vi "CreateClass.vi"(0 "ClassWriterGOOP300.lvclass":refnum<class "ClassWriterGOOP300.lvclass">, 1 "ProjectTreePosition(String or Project Item Ref)":variant, 2 "CreateClassData":T1, 5 "error in (no error)":errorcluster, 6 "KeepLvClassRefOpen(False)":bool, 7 "HeaderToApply (take from VIRef or /use 2D-8bit header, Ignored if not wired)":variant) -> (14 "ClassWriterGOOP300.lvclass":refnum<class "ClassWriterGOOP300.lvclass">, 15 "LVClassLibraryRefnum":refnum<vi>, 16 "TemplateVersionUsed":string, 19 "error out":errorcluster)   [LabVIEW 2020, in "ClassWriterGOOP300.lvclass"]
uses:
  ClassWriterGOOP300.lvclass
  Provider_BaseClassInterface/CreateClassData.ctl
  Common/LvClass_class/GDSLvCLass_ClassSettingsType.ctl
  Common/LvClass_class/GDSLvClass_PlugIn.ctl
  Common/LvClass_class/GDSLvClass_PlugInTypes.ctl
  Provider_EndevoGOOP400/EndevoG4ProviderName.ctl
  EndevoProviderName.ctl
  Provider_BaseClassInterface/ClassWriter_class/ClassWriter.lvclass
  Provider_LvNativeClass/ClassWriterNative_class/ClassWriterNative.lvclass
  Provider_EndevoGOOP400/ClassWriterGOOP400_class/ClassWriterGOOP400.lvclass
  Common/InterfaceLibrary/InterfaceLibrary.lvlib
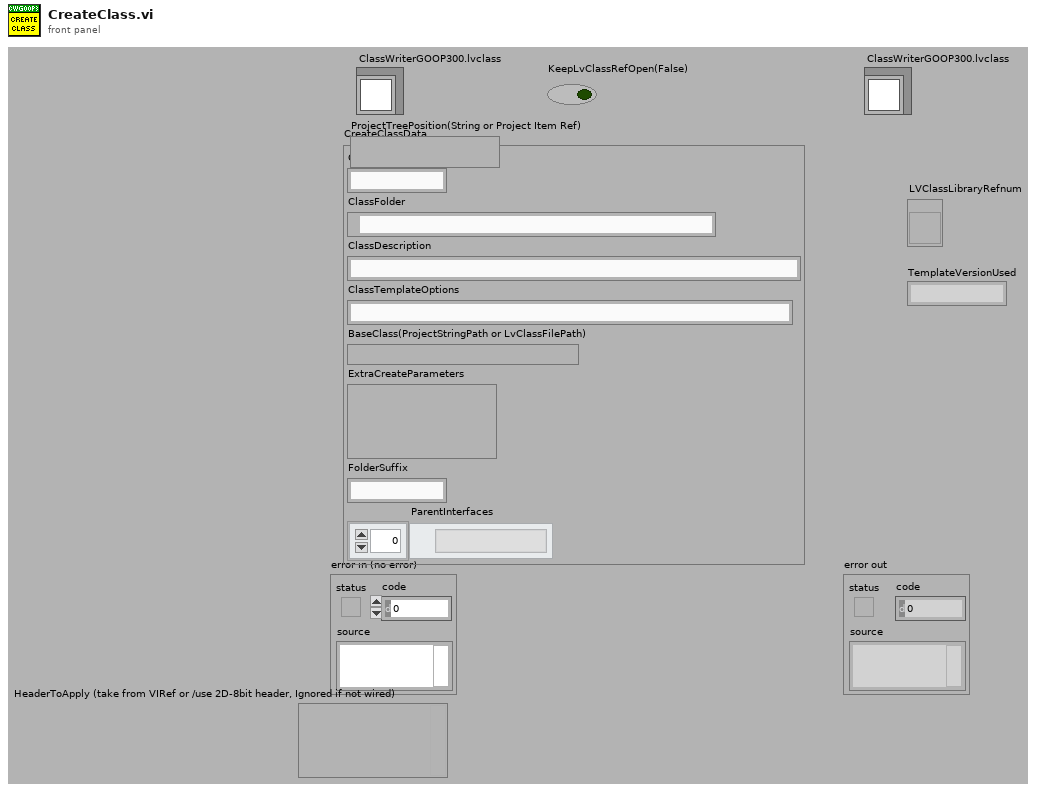
[diagram p1: front panel]
types:
  T1 = typedef "ClassWriter.lvclass/CreateClassData.ctl" = cluster{"ClassName":string, "ClassFolder":path, "ClassDescription":string, "ClassTemplateOptions":string, "BaseClass(ProjectStringPath or LvClassFilePath)":variant, "ExtraCreateParameters":variant, "FolderSuffix":string, "ParentInterfaces":path[]}
  T2 = typedef "GDSLvCLass_ClassSettingsType.ctl" = cluster{"ClassProviderName":string, "ClassTemplateUsed":string, "ClassTemplateVersion":string, "ClassDescription":string, "PlugIns":T3[], "ConnectorPanePattern":string}
  T3 = typedef "GDSLvClass_PlugIn.ctl" = cluster{"Type":T4, "ID":string, "Version":string, "Path":path, "Name":string, "Data":variant}
  T4 = typedef "GDSLvClass_PlugInTypes.ctl" = enum16{"DesignPattern", "MethodTypes"}
  T5 = cluster{"SubClass":bool, "ClassTemplateFiles":path[], "ClassName":string, "ClassFolder":path, "VIs":refnum<vi>[], "TemplateFolder":path, "ViSubDirs":string[], "TemplateName":string, "BaseClassFolder":path, "RootBaseClassFolder":path, "LvClassPath":path, "ClassRefnum":refnum<vi>, "ProjectRefnum":refnum<vi>, "LvClassFolderPath":path, "BaseClassName":string, "ClassItems":refnum<vi>[], "ViLocked":bool[], "ProjectItemOwner":refnum<vi>, "DeleteFiles":path[], "VIsBefore":refnum<vi>[], "BaseClassPath":path, "BaseConstructorBase":path, "TemplBaseConstructorBase":path, "TemplatePath":path, "TemplateVersion":string, "TemplateParentClass":refnum<vi>, "App":refnum<vi>, "Parent Class":refnum<vi>, "ParentVIs":refnum<vi>[], "TempClass":refnum<vi>, "TemplateParentName":string, "llb":bool, "ClassSettings":T2}
  T6 = typedef "EndevoG4ProviderName.ctl" = enum16{"EndevoGOOP400"}
  T7 = typedef "EndevoProviderName.ctl" = enum16{"EndevoGOOP300"}
  T8 = enum32{"invalid scope", "public", "private", "protected"}
  T9 = enum16{"Share clones between instances", "Preallocate clone for each instance"}
  T10 = enum32{"invalid lock state", "Not Locked", "Locked (No Password)", "Password-protected"}
  T11 = typedef "ClassWriter.lvclass/TemplateSettings.ctl" = cluster{"CommonClassTemplate":bool, "DynamicDispatch":enum8{"False", "True", "Mixed"}, "MustOverride":enum8{"False", "True", "Mixed"}, "MustCallParent":enum8{"False", "True", "Mixed"}, "OnlyNormalMethod":bool, "OnlyPublic":bool}
  T12 = typedef "Scripting_ConnectorPanePatternType.ctl" = u16
  T13 = typedef "GOOP400_Options.ctl" = cluster{"FlatFolderStructure":bool}
  T14 = typedef "imagedata.ctl" = cluster{"image type":i32, "image depth":i32, "image":u8[], "mask":u8[], "colors":u32[], "Rectangle":cluster{"left":i16, "top":i16, "right":i16, "bottom":i16}}
  T15 = typedef "Librarian File Info Out.ctl" = cluster{"creation date":u32, "last mod date":u32, "type":string, "creator":string, "LV version":i32, "size":i32, "top level":bool}
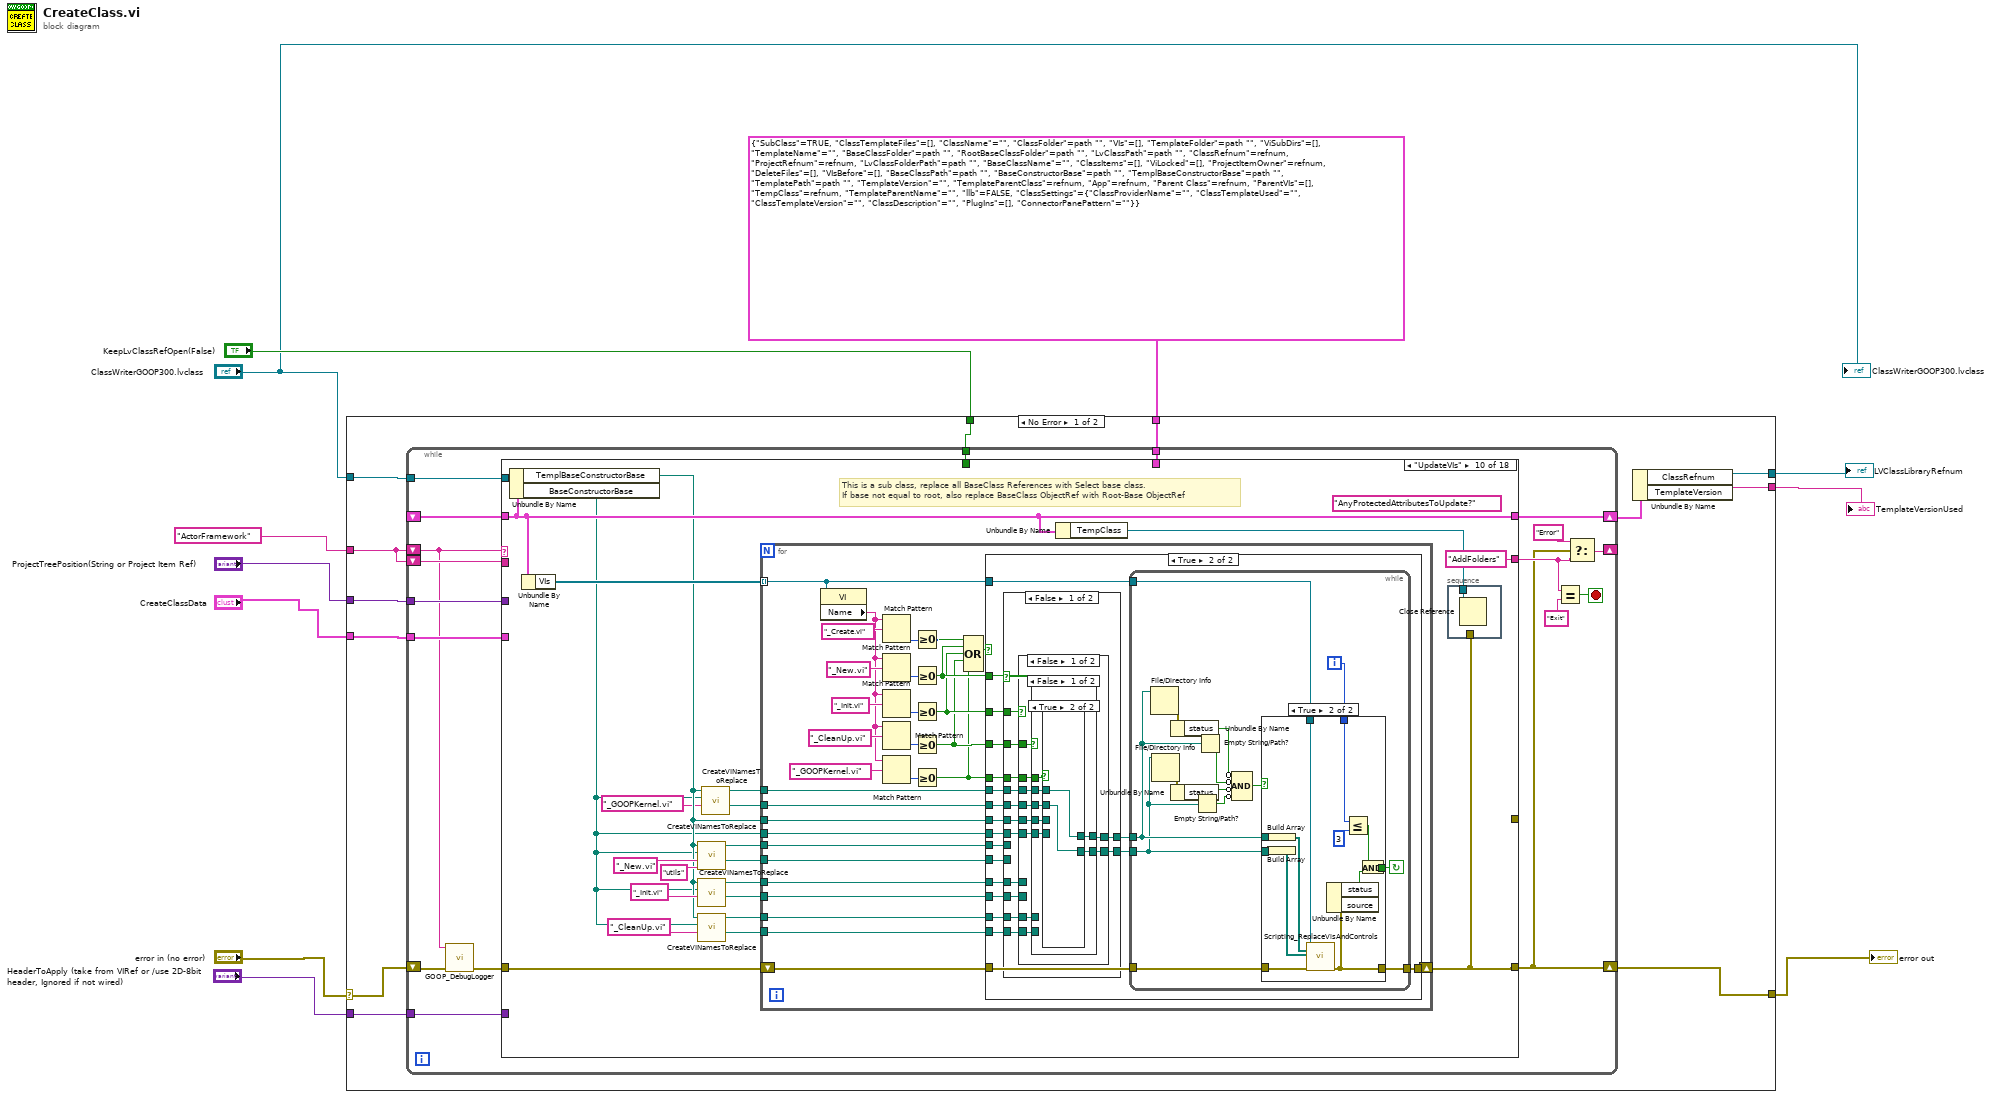
[diagram p0: block diagram]
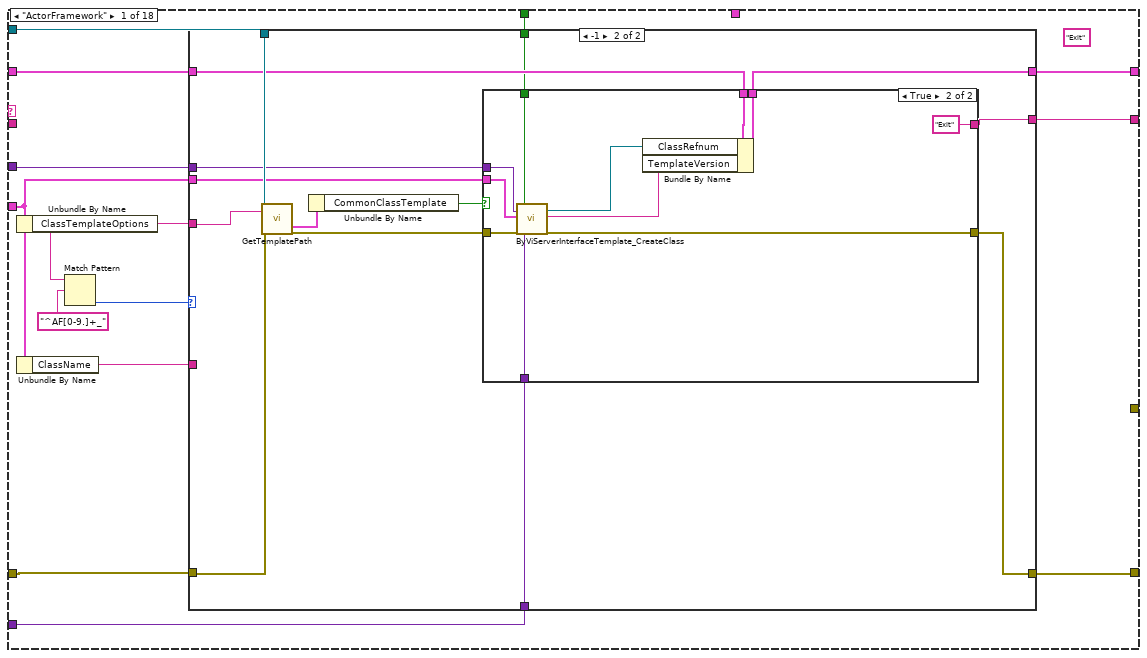
[diagram p2: hidden frame]
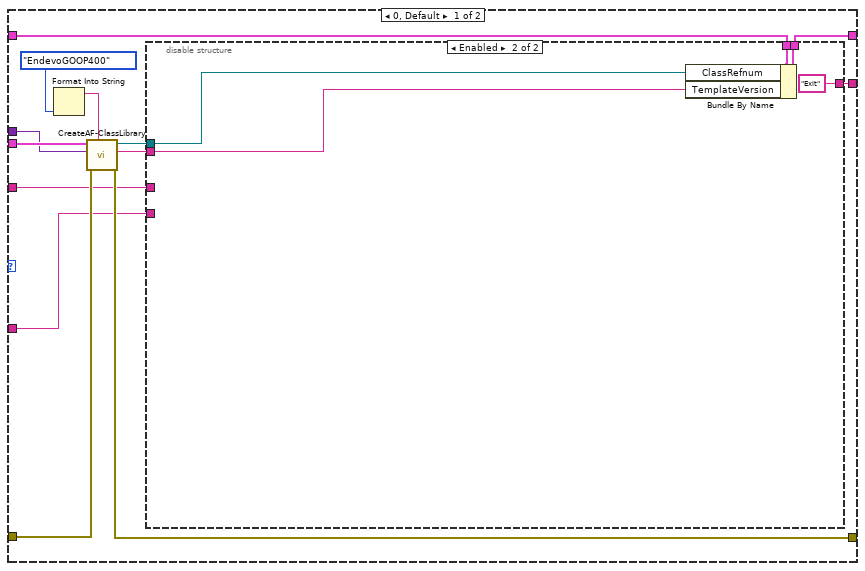
[diagram p3: hidden frame]
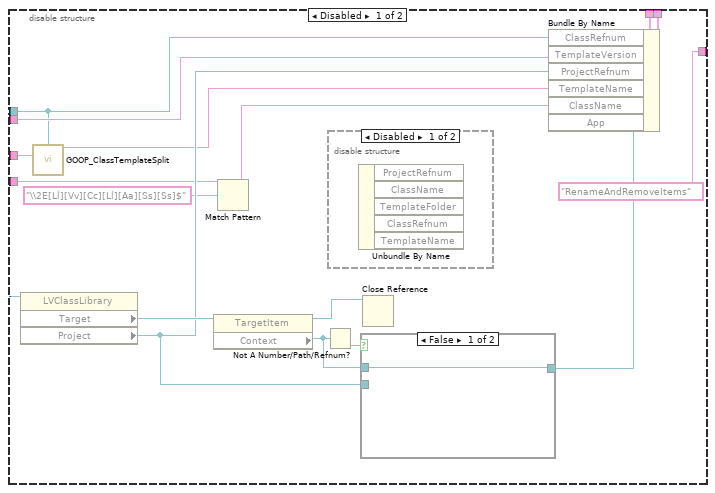
[diagram p4: hidden frame]
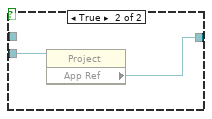
[diagram p6: hidden frame]
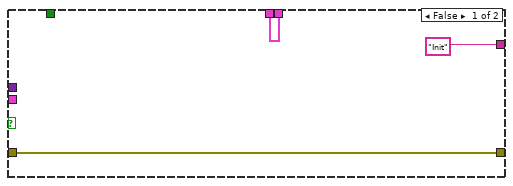
[diagram p7: hidden frame]
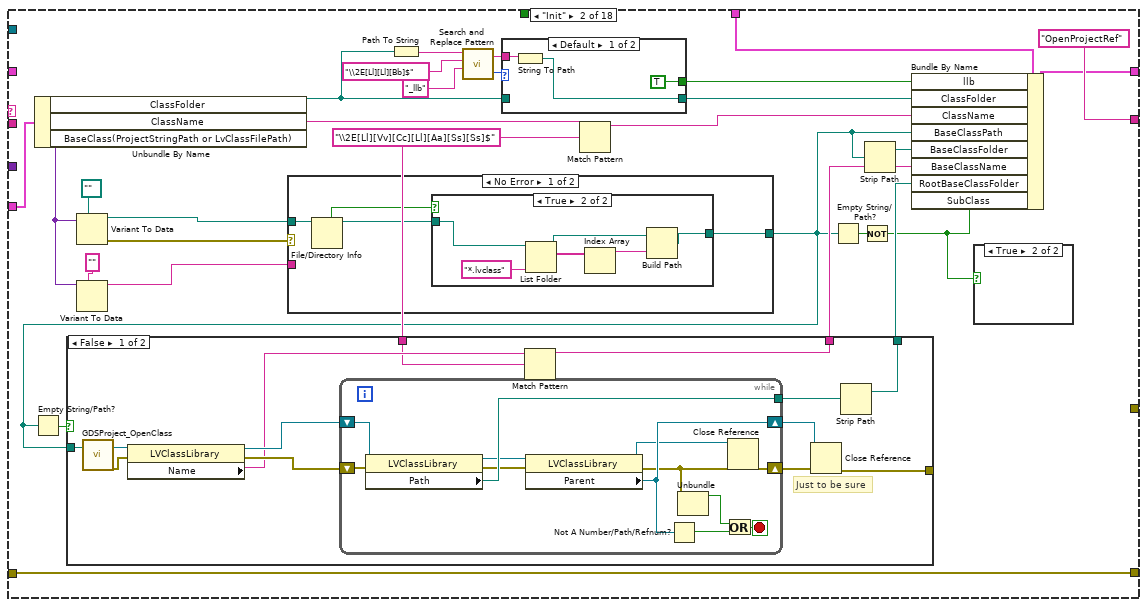
[diagram p8: hidden frame]
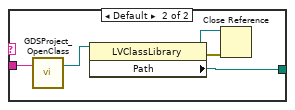
[diagram p14: hidden frame]
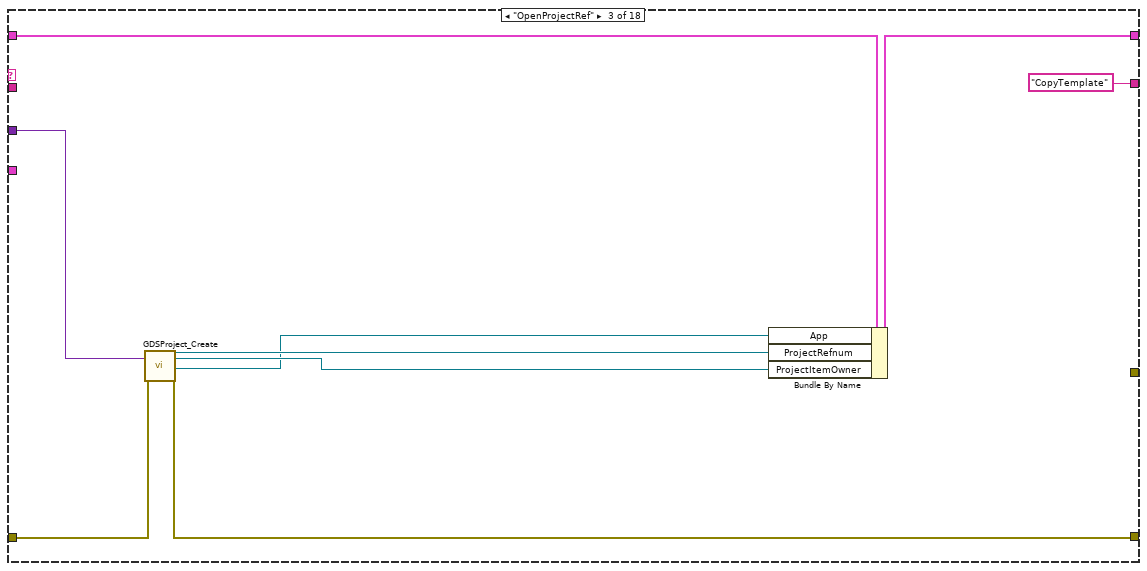
[diagram p15: hidden frame]
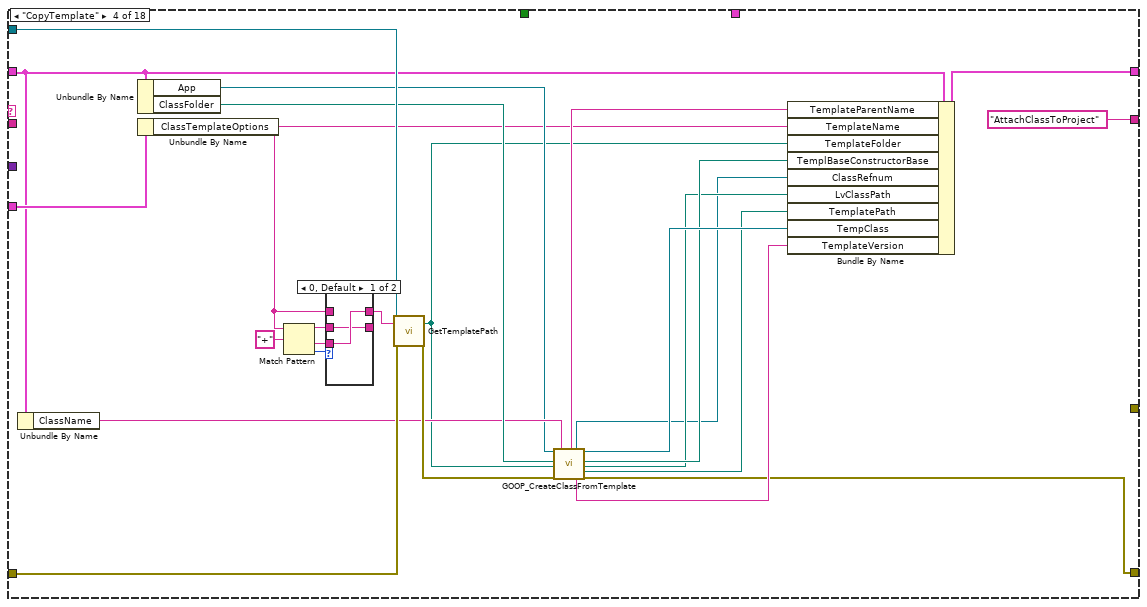
[diagram p16: hidden frame]
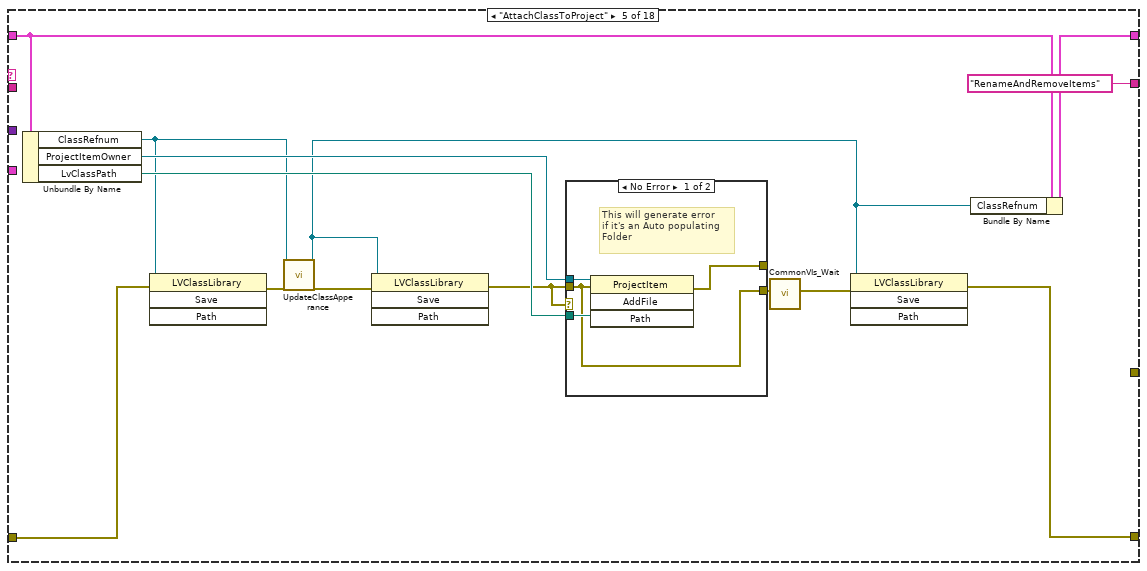
[diagram p18: hidden frame]
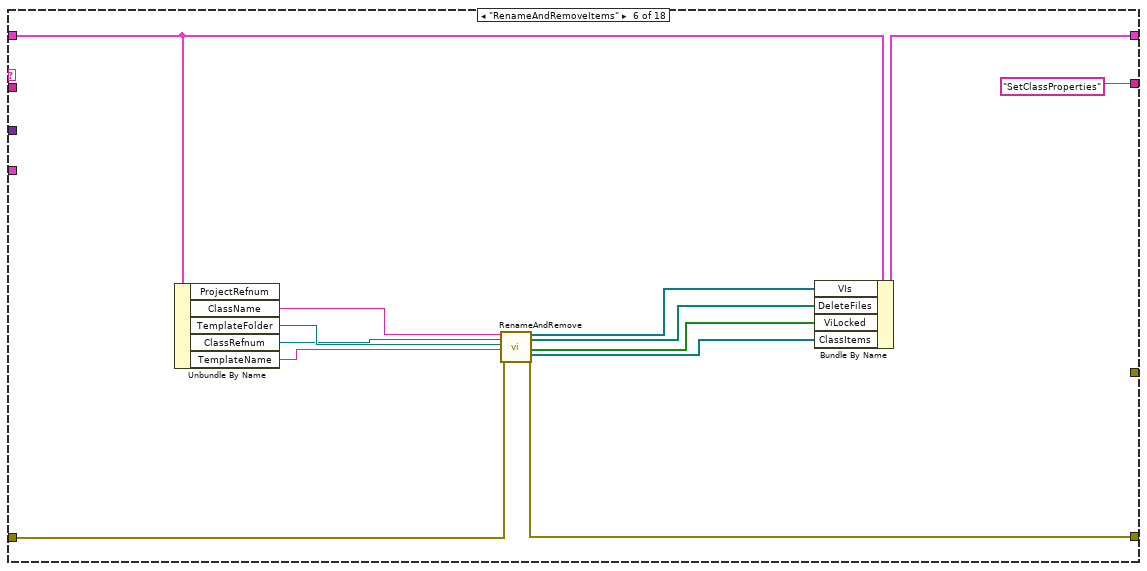
[diagram p20: hidden frame]
diagram:
  n1 = case shown="No Error" "error in (no error)" {
    selector: "error in (no error)" -> [w13 w824]
    tunnel: [w23 w824] -> w11
    tunnel: "ProjectTreePosition(String or Project Item Ref)" -> [w22 _]
    tunnel: "CreateClassData" -> [w21 _]
    tunnel: "ClassWriterGOOP300.lvclass" -> [w20 _]
    tunnel: "HeaderToApply (take from VIRef or /use 2D-8bit header, Ignored if not wired)" -> [w19 _]
    tunnel: "KeepLvClassRefOpen(False)" -> [w18 _]
    tunnel: [w17 _] -> w5
    tunnel: [w16 _] -> w4
    tunnel: T5 {"SubClass"=TRUE, "ClassTemplateFiles"=[], "ClassName"="", "ClassFolder"=path "", "VIs"=[], "TemplateFolder"=path "", "ViSubDirs"=[], "TemplateName"="", "BaseClassFolder"=path "", "RootBaseClassFolder"=path "", "LvClassPath"=path "", "ClassRefnum"=refnum, "ProjectRefnum"=refnum, "LvClassFolderPath"=path "", "BaseClassName"="", "ClassItems"=[], "ViLocked"=[], "ProjectItemOwner"=refnum, "DeleteFiles"=[], "VIsBefore"=[], "BaseClassPath"=path "", "BaseConstructorBase"=path "", "TemplBaseConstructorBase"=path "", "TemplatePath"=path "", "TemplateVersion"="", "TemplateParentClass"=refnum, "App"=refnum, "Parent Class"=refnum, "ParentVIs"=[], "TempClass"=refnum, "TemplateParentName"="", "llb"=FALSE, "ClassSettings"={"ClassProviderName"="", "ClassTemplateUsed"="", "ClassTemplateVersion"="", "ClassDescription"="", "PlugIns"=[], "ConnectorPanePattern"=""}} ("output cluster") -> [w15 _]
    tunnel: "ActorFramework" -> [w12 _]
    frame No Error {
      n2 = while {
        shift-right: [w33] -> w23
        shift-left: w13 -> [w26]
        shift-right: [w37] -> _
        shift-left: w12 -> [w24]
        shift-right: [w40] -> w14
        shift-left: _ -> [w41]
        tunnel: w15 -> [w35]
        tunnel: w22 -> [w32]
        tunnel: w21 -> [w31]
        tunnel: w20 -> [w30]
        shift-left: w12 -> [w29]
        tunnel: w19 -> [w28]
        tunnel: w18 -> [w27]
        stop <- w38 stop-if-true
        n3 = call "GOOP_DebugLogger.vi"("error in (no error)"=w26, "State"=w24) -> ("error out"=w25:errorcluster)  [unwired: 7 in, 2 out]
        n4 = case shown="\"UpdateVIs\"" w24 {
          selector: w24 -> [_ _ _ _ _ _ _ _ _ _ _ _ _ _ _ _ _ w775]
          tunnel: w41 -> [w55 _ w203 w214 w245 w260 w278 w328 w350 w364 w497 w554 w591 w643 w669 w680 w728 w759]
          tunnel: [w54 w146 w202 w213 w244 w262 w267 w328 w351 w364 w497 w554 w591 w643 w669 w680 w728 w759] -> w40
          tunnel: w25 -> [w50 w149 w201 w226 w239 w257 w279 w321 w347 w376 w518 w566 w592 w647 w668 w681 w731 w776]
          tunnel: [w49 w149 w199 w211 w235 w258 w270 w318 w333 w362 w498 w567 w593 w648 w667 w681 w714 w772] -> w33
          tunnel: [w53 "OpenProjectRef" "CopyTemplate" "AttachClassToProject" "RenameAndRemoveItems" "SetClassProperties" "UpdateIcons" w330 "UpdateVIs" ("t") "AddFolders" "AddFolders" w553 "PlaceRefInAttribute" "PlaceRefInAttribute" "ReentrantDestructor?" w685 "CloseRefs" "Exit"] -> w34
          tunnel: w35 -> [_ w142 _ _ _ _ _ _ _ _ _ _ _ _ _ _ _ _]
          tunnel: w32 -> [w48 _ w200 _ _ _ _ _ _ _ _ _ _ _ _ _ _ _]
          tunnel: w31 -> [w46 w141 _ w228 _ _ w285 _ _ _ _ w552 _ _ _ _ w733 _]
          tunnel: w30 -> [w44 _ _ w227 _ _ _ w315 _ _ _ _ _ w649 _ _ _ _]
          tunnel: w29 -> [_ _ _ _ _ _ _ _ _ _ _ _ _ _ _ _ _ w771]
          tunnel: w28 -> [w42 _ _ _ _ _ _ w326 _ _ _ _ _ _ _ _ _ _]
          tunnel: w27 -> [w43 _ _ _ _ _ _ _ _ _ _ _ _ _ _ _ _ w767]
          tunnel: [_ _ _ _ _ _ _ _ _ _ _ _ _ _ _ _ _ w765] -> _
          frame "ActorFramework" {
            (unwired) "Exit"
            n5 = Unbundle By Name(w46) -> ("ClassTemplateOptions"=w47:string)
            n6 = Unbundle By Name(w46) -> ("ClassName"=w45:string)
            n7 = Match Pattern(string=w47, regular expression="^AF[0-9.]+_") -> (offset past match=w51:i32)  [unwired: 1 in, 3 out]
            n8 = case shown="-1" w51 {
              tunnel: w55 -> [w68 w100]
              tunnel: [w67 w99] -> w54
              tunnel: [w59 w106] -> w53
              tunnel: w46 -> [w65 w96]
              tunnel: w50 -> [w64 w104]
              tunnel: [w63 w101] -> w49
              tunnel: w48 -> [w60 w97]
              tunnel: w47 -> [w57 w103]
              tunnel: w45 -> [w56 _]
              tunnel: w44 -> [_ w105]
              tunnel: w43 -> [_ w98]
              tunnel: w42 -> [_ w95]
              frame 0, Default {
                n9 = Format Into String(EndevoG4ProviderName."EndevoGOOP400" ("ProviderName")) -> (resulting string=w62:string)  [unwired: 3 in, 1 out]
                n10 = call "CreateAF-ClassLibrary.vi"("Providername"=w62, "error in (no error)"=w64, "ProjectTreePosition(String or Project Item Ref)"=w60, "CreateClassData"=w65) -> ("error out"=w63:errorcluster, "TemplateVersionUsed"=w61:string, "LVClassLibraryRefnum"=w58:refnum<vi>)  [unwired: 5 in]
                n11 = disable-structure shown="Enabled" {
                  disable-tunnel: w68 -> [w84 w92]
                  disable-tunnel: [w83 w91] -> w67
                  disable-tunnel: w61 -> [w82 w89]
                  disable-tunnel: ["RenameAndRemoveItems" "Exit"] -> w59
                  disable-tunnel: w58 -> [w74 w90]
                  disable-tunnel: w57 -> [w73 _]
                  disable-tunnel: w56 -> [w70 _]
                  frame Disabled {
                    n12 = property class="LVClassLibrary"(reference=w74) -> ("Target"=w80:refnum<vi>, "Project"=w75:refnum<vi>)  [unwired: 1 in, 2 out]
                    n13 = call "GOOP_ClassTemplateSplit.vi"("ClassItemRefIn"=w74, "FullClassTemplate"=w73) -> ("StandardTemplate"=w72:string)  [unwired: 12 in, 1 out]
                    n14 = property class="TargetItem"(reference=w80) -> (reference out=w79:refnum<vi>, "Context"=w77:refnum<vi>)  [unwired: 1 in, 1 out]
                    n15 = Match Pattern(string=w70, regular expression="\\2E[Ll][Vv][Cc][Ll][Aa][Ss][Ss]$") -> (before substring=w69:string)  [unwired: 1 in, 3 out]
                    n16 = Not A Number/Path/Refnum?(number/path/refnum=w77) -> (NaN/Path/Refnum?=w78:bool)
                    n17 = disable-structure shown="Disabled" {
                      frame Disabled {
                        n18 = Unbundle By Name() -> ()  [unwired: 1 in, 5 out]
                      }
                      frame Enabled {
                      }
                    }
                    n19 = case shown="False" w78 {
                      tunnel: [w85 w86] -> w76
                      tunnel: w75 -> [_ w87]
                      tunnel: w77 -> [w85 _]
                      frame False {
                      }
                      frame True {
                        n20 = property class="Project"(reference=w87) -> ("App Ref"=w86:refnum<vi>)  [unwired: 1 in, 2 out]
                      }
                    }
                    n21 = Close Reference(reference=w79) -> ()  [unwired: 1 in, 1 out]
                    n22 = Bundle By Name(cluster=w84, "ClassRefnum"=w74, "TemplateVersion"=w82, "ProjectRefnum"=w75, "TemplateName"=w72, "ClassName"=w69, "App"=w76) -> (w83:T5)
                  }
                  frame Enabled {
                    n23 = Bundle By Name(cluster=w92, "ClassRefnum"=w90, "TemplateVersion"=w89) -> (w91:T5)
                  }
                }
              }
              frame -1 {
                n24 = call-dynamic "GetTemplatePath.vi"("reference in"=w105, "ClassTemplateSubDirectory"=w103, "error in (no error)"=w104) -> ("TemplateSettings"=w94:T11, "error out"=w102:errorcluster)  [unwired: 12 in, 3 out]
                n25 = Unbundle By Name(w94) -> ("CommonClassTemplate"=w93:bool)
                n26 = case shown="True" w93 {
                  tunnel: ["Init" "Exit"] -> w106
                  tunnel: w102 -> [w107 w117]
                  tunnel: [w107 w116] -> w101
                  tunnel: w100 -> [w108 w115]
                  tunnel: [w108 w114] -> w99
                  tunnel: w98 -> [_ w113]
                  tunnel: w97 -> [_ w112]
                  tunnel: w96 -> [_ w111]
                  tunnel: w95 -> [_ w110]
                  frame False {
                  }
                  frame True {
                    n27 = call "ByViServerInterfaceTemplate_CreateClass.vi"("ProjectTreePosition(String or Project Item Ref)"=w112, "CreateClassData"=w111, "error in (no error)"=w117, "KeepLvClassRefOpen(False)"=w113, "HeaderToApply (take from VIRef or /use 2D-8bit header, Ignored if not wired)"=w110) -> ("LVClassLibraryRefnum"=w119:refnum<vi>, "TemplateVersionUsed"=w118:string, "error out"=w116:errorcluster)  [unwired: 12 in]
                    n28 = Bundle By Name(cluster=w115, "ClassRefnum"=w119, "TemplateVersion"=w118) -> (w114:T5)
                  }
                }
              }
            }
          }
          frame "Init" {
            w138 = "\\2E[Ll][Vv][Cc][Ll][Aa][Ss][Ss]$" ("regular expression")
            n29 = Unbundle By Name(w141) -> ("ClassFolder"=w124:path, "ClassName"=w135:string, "BaseClass(ProjectStringPath or LvClassFilePath)"=w140:variant)
            n30 = Variant To Data(type=path "" ("path"), Variant=w140) -> (data=w132:path, error out=w133:errorcluster)  [unwired: 1 in]
            n31 = Variant To Data(type="" ("regular expression"), Variant=w140) -> (data=w143:string)  [unwired: 1 in, 1 out]
            n32 = case shown="No Error" w133 {
              tunnel: [w181 w189] -> w130
              tunnel: w143 -> [_ w190]
              tunnel: w132 -> [w180 _]
              frame No Error {
                n33 = File/Directory Info(path=w180) -> (path out=w178:path, directory=w179:bool)  [unwired: 1 in, 5 out]
                n34 = case shown="True" w179 {
                  tunnel: [w182 w184] -> w181
                  tunnel: w178 -> [w182 w183]
                  frame False {
                  }
                  frame True {
                    n35 = List Folder(path=w183, pattern="*.lvclass") -> (path out=w185:path, filenames=w187:string[])  [unwired: 2 in, 2 out]
                    n36 = Index Array(array=w187) -> (element=w186:string)  [unwired: 1 in]
                    n37 = Build Path(base path=w185, name or relative path=w186) -> (appended path=w184:path)
                  }
                }
              }
              frame Error {
                n38 = case shown="\"\"" w190 {
                  tunnel: w190 -> [_ w195]
                  tunnel: [_ w191] -> w189
                  frame "" {
                  }
                  frame Default {
                    n39 = call "GDSProject_OpenClass.vi"("ClassPath(FilePath/ProjectTreePath/LvCLassRef)"=w195) -> ("LVClass.Open"=w194:refnum<vi>)  [unwired: 16 in, 2 out]
                    n40 = property class="LVClassLibrary"(reference=w194) -> (reference out=w192:refnum<vi>, error out=w193:errorcluster, "Path"=w191:path)  [unwired: 1 in]
                    n41 = Close Reference(reference=w192, error in (no error)=w193) -> ()  [unwired: 1 out]
                  }
                }
              }
            }
            n42 = Empty String/Path?(string/path=w130) -> (empty?=w136:bool)
            n43 = case shown="False" w136 {
              tunnel: [w163 _] -> w139
              tunnel: w138 -> [w157 _]
              tunnel: [w156 _] -> w137
              tunnel: w130 -> [w155 _]
              tunnel: [w154 _] -> _
              frame False {
                # "Just to be sure"
                n44 = call "GDSProject_OpenClass.vi"("ClassPath(FilePath/ProjectTreePath/LvCLassRef)"=w155) -> ("LVClass.Open"=w160:refnum<vi>, "error out"=w162:errorcluster)  [unwired: 16 in, 1 out]
                n45 = property class="LVClassLibrary"(reference=w160, error in=w162) -> (reference out=w159:refnum<vi>, error out=w161:errorcluster, "Name"=w158:string)
                n46 = while {
                  shift-right: [w174] -> w166
                  shift-left: w161 -> [w169]
                  shift-right: [w175] -> w165
                  shift-left: w159 -> [w177]
                  tunnel: [w176] -> w164
                  stop <- w171 stop-if-true
                  n47 = property class="LVClassLibrary"(reference=w177, error in=w169) -> (reference out=w167:refnum<vi>, error out=w168:errorcluster, "Path"=w176:path)
                  n48 = property class="LVClassLibrary"(reference=w167, error in=w168) -> (reference out=w170:refnum<vi>, error out=w174:errorcluster, "Parent"=w175:refnum<vi>)
                  n49 = Not A Number/Path/Refnum?(number/path/refnum=w175) -> (NaN/Path/Refnum?=w172:bool)
                  n50 = Unbundle(w174) -> ("status"=w173:bool)  [unwired: 2 out]
                  n51 = Or(x=w173, y=w172) -> (x .or. y?=w171:bool)
                  n52 = Close Reference(reference=w170) -> ()  [unwired: 1 in, 1 out]
                }
                n53 = Match Pattern(string=w158, regular expression=w157) -> (before substring=w156:string)  [unwired: 1 in, 3 out]
                n54 = Close Reference(reference=w165, error in (no error)=w166) -> (error out=w154:errorcluster)
                n55 = Strip Path(path=w164) -> (stripped path=w163:path)  [unwired: 1 out]
              }
              frame True {
              }
            }
            n56 = Path To String(path=w124) -> (string=w128:string)
            n57 = call <vilib>:"Search and Replace Pattern.vi"("string"=w128, "regular expression (\"\")"="\\2E[Ll][Ll][Bb]$" ("regular expression (\"\")"), "replace string (\"\")"="_llb" ("replace string (\"\")")) -> ("result string"=w121:string, "offset past match"=w126:i32)  [unwired: 2 in]
            n58 = case shown="Default" w126 {
              tunnel: w124 -> [_ w153]
              tunnel: [w150 w153] -> w123
              tunnel: [TRUE _] -> w122
              tunnel: w121 -> [w151 _]
              frame Default {
                n59 = String To Path(string=w151) -> (path=w150:path)
              }
              frame -1 {
              }
            }
            n60 = Match Pattern(string=w135, regular expression=w138) -> (before substring=w147:string)  [unwired: 1 in, 3 out]
            n61 = Empty String/Path?(string/path=w130) -> (empty?=w131:bool)
            n62 = Not(x=w131) -> (.not. x?=w129:bool)
            n63 = Strip Path(path=w130) -> (stripped path=w134:path)  [unwired: 1 out]
            n64 = Bundle By Name(cluster=w142, "llb"=w122, "ClassFolder"=w123, "ClassName"=w147, "BaseClassPath"=w130, "BaseClassFolder"=w134, "BaseClassName"=w137, "RootBaseClassFolder"=w139, "SubClass"=w129) -> (w146:T5)
            n65 = case shown="True" w129 {
              frame False {
              }
              frame True {
              }
            }
          }
          frame "OpenProjectRef" {
            n66 = call "GDSProject_Create.vi"("ProjectTreePosition(String or Project Item Ref)"=w200, "error in (no error)"=w201) -> ("Project Refnum"=w197:refnum<vi>, "Project Item"=w198:refnum<vi>, "App"=w196:refnum<vi>, "error out"=w199:errorcluster)  [unwired: 13 in, 1 out]
            n67 = Bundle By Name(cluster=w203, "App"=w196, "ProjectRefnum"=w197, "ProjectItemOwner"=w198) -> (w202:T5)
          }
          frame "CopyTemplate" {
            n68 = Unbundle By Name(w214) -> ("ClassName"=w208:string)
            n69 = Unbundle By Name(w214) -> ("App"=w207:refnum<vi>, "ClassFolder"=w209:path)
            n70 = Unbundle By Name(w228) -> ("ClassTemplateOptions"=w206:string)
            n71 = Match Pattern(string=w206, regular expression="+") -> (before substring=w222:string, after substring=w225:string, offset past match=w224:i32)  [unwired: 1 in, 1 out]
            n72 = case shown="0, Default" w224 {
              tunnel: w206 -> [_ w232]
              tunnel: [w231 w232] -> w221
              tunnel: w225 -> [w231 _]
              tunnel: [w230 _] -> _
              tunnel: w222 -> [w230 _]
              frame 0, Default {
              }
              frame -1 {
              }
            }
            n73 = call-dynamic "GetTemplatePath.vi"("reference in"=w227, "ClassTemplateSubDirectory"=w221, "error in (no error)"=w226) -> ("FolderPathOut"=w205:path, "error out"=w210:errorcluster)  [unwired: 12 in, 3 out]
            n74 = call "GOOP_CreateClassFromTemplate.vi"("Application in"=w207, "ClassFolder"=w209, "TeplateClassFolder"=w205, "error in (no error)"=w210, "ClassName"=w208) -> ("TemplateParentName"=w212:string, "NewClassRef"=w217:refnum<vi>, "TemplateClassVersionString"=w215:string, "TemplateClassRef"=w220:refnum<vi>, "TemplateClassConstructorPath(*Create, *Init)"=w219:path, "NewClassPath"=w218:path, "TemplateClassPath"=w216:path, "error out"=w211:errorcluster)  [unwired: 7 in]
            n75 = Bundle By Name(cluster=w214, "TemplateParentName"=w212, "TemplateName"=w206, "TemplateFolder"=w205, "TemplBaseConstructorBase"=w219, "ClassRefnum"=w217, "LvClassPath"=w218, "TemplatePath"=w216, "TempClass"=w220, "TemplateVersion"=w215) -> (w213:T5)
          }
          frame "AttachClassToProject" {
            n76 = Unbundle By Name(w245) -> ("ClassRefnum"=w238:refnum<vi>, "ProjectItemOwner"=w246:refnum<vi>, "LvClassPath"=w242:path)
            n77 = invoke class="LVClassLibrary" method="Save"(reference=w238, error in=w239) -> (error out=w240:errorcluster)  [unwired: 2 in, 3 out]
            n78 = call "UpdateClassApperance.vi"("ClassRefIn"=w238, "error in (no error)"=w240) -> ("ClassRefOut"=w233:refnum<vi>, "error out"=w237:errorcluster)  [unwired: 16 in]
            n79 = invoke class="LVClassLibrary" method="Save"(reference=w233, error in=w237) -> (error out=w234:errorcluster)  [unwired: 2 in, 3 out]
            n80 = case shown="No Error" w234 {
              tunnel: w246 -> [w250 _]
              tunnel: w242 -> [w249 _]
              tunnel: [w248 w251] -> w241
              tunnel: w234 -> [w248 w251]
              tunnel: [w247 _] -> _
              frame No Error {
                # "This will generate error\nif it's an Auto populating\nFolder"
                n81 = invoke class="ProjectItem" method="AddFile"(reference=w250, error in=w248, "Path"=w249) -> (error out=w247:errorcluster)  [unwired: 1 in, 3 out]
              }
              frame Error {
              }
            }
            n82 = call "CommonVIs_Wait.vi"("error in"=w241) -> ("error out"=w236:errorcluster)  [unwired: 9 in]
            n83 = invoke class="LVClassLibrary" method="Save"(reference=w233, error in=w236) -> (error out=w235:errorcluster)  [unwired: 2 in, 3 out]
            n84 = Bundle By Name(cluster=w245, "ClassRefnum"=w233) -> (w244:T5)
          }
          frame "RenameAndRemoveItems" {
            n85 = Unbundle By Name(w260) -> ("ClassName"=w264:string, "TemplateFolder"=w261:path, "ClassRefnum"=w259:refnum<vi>, "TemplateName"=w252:string)  [unwired: 1 out]
            n86 = call "RenameAndRemove.vi"("ClassName"=w264, "ClassRefnum"=w259, "TemplateFolder"=w261, "TemplateName"=w252, "error in"=w257) -> ("ViRefsOut"=w263:refnum<vi>[], "DeleteFiles"=w256:path[], "ItemLocked"=w255:bool[], "Items"=w254:refnum<vi>[], "error out"=w258:errorcluster)  [unwired: 10 in]
            n87 = Bundle By Name(cluster=w260, "VIs"=w263, "DeleteFiles"=w256, "ViLocked"=w255, "ClassItems"=w254) -> (w262:T5)
          }
          frame "SetClassProperties" {
            n88 = Unbundle By Name(w285) -> ("ClassDescription"=w282:string)
            n89 = Unbundle By Name(w278) -> ("ClassRefnum"=w280:refnum<vi>, "App"=w275:refnum<vi>)
            n90 = Unbundle By Name(w278) -> ("TemplateName"=w281:string, "TemplateVersion"=w276:string, "SubClass"=w289:bool)
            n91 = Unbundle By Name(w278) -> ("BaseClassPath"=w288:path)
            n92 = case shown="False" w289 {
              tunnel: w280 -> [w297 w314]
              tunnel: [w308 w314] -> w287
              tunnel: w279 -> [w301 w310]
              tunnel: [w307 w309] -> w286
              tunnel: w288 -> [w306 _]
              tunnel: w275 -> [w302 _]
              tunnel: [w303 w311] -> w274
              tunnel: [w295 _] -> w269
              frame True {
                n93 = invoke class="LVClassLibrary" method="Save"(reference=w297) -> (reference out=w296:refnum<vi>)  [unwired: 3 in, 3 out]
                n94 = invoke class="App" method="LVClass.Open"(reference=w302, error in=w301, "Path"=w306) -> (error out=w300:errorcluster, "LVClass.Open"=w305:refnum<vi>)  [unwired: 1 in, 2 out]
                n95 = call "CommonVIs_Wait.vi"("error in"=w300) -> ("error out"=w299:errorcluster)  [unwired: 9 in]
                n96 = call "GDSLvClass_ReadClassType.vi"("Class Refnum In"=w305, "error in (no error)"=w299) -> ("Class Refnum Out"=w295:refnum<vi>, "ClassSettings"=w304:T2, "error out"=w298:errorcluster)  [unwired: 15 in]
                n97 = Unbundle By Name(w304) -> ("ConnectorPanePattern"=w303:string)
                n98 = invoke class="LVClassLibrary" method="Save"(reference=w295) -> (reference out=w294:refnum<vi>)  [unwired: 3 in, 3 out]
                n99 = property class="LVClassLibrary"(reference=w296, error in=w298, "Parent"=w294) -> (reference out=w308:refnum<vi>, error out=w307:errorcluster)
              }
              frame False {
                n100 = call "BaseProvider_ConfigurationMemory.vi"("error in (no error)"=w310, "Action"=enum16{"Read", "Load", "Save"}."Read") -> ("PatternOut"=w313:T12, "error out"=w309:errorcluster)  [unwired: 11 in, 5 out]
                n101 = Format Into String(w313) -> (resulting string=w311:string)  [unwired: 3 in, 1 out]
              }
            }
            n102 = Format Into String(EndevoProviderName."EndevoGOOP300" ("ProviderName")) -> (resulting string=w283:string)  [unwired: 3 in, 1 out]
            n103 = Bundle By Name(cluster=T2 {"ClassProviderName"="", "ClassTemplateUsed"="", "ClassTemplateVersion"="", "ClassDescription"="", "PlugIns"=[], "ConnectorPanePattern"=""} ("ClassSettings"), "ClassProviderName"=w283, "ClassTemplateUsed"=w281, "ClassTemplateVersion"=w276, "ClassDescription"=w282, "ConnectorPanePattern"=w274) -> (w266:T2)
            n104 = Bundle By Name(cluster=w278, "ClassSettings"=w266) -> (w267:T5)
            n105 = call "GDSLvClass_StoreClassType.vi"("Class Refnum In"=w287, "ClassSettings"=w266, "CheckAndFixConnectorPaneType(False)"=TRUE, "error in (no error)"=w286) -> ("Class Refnum Out"=w273:refnum<vi>, "error out"=w272:errorcluster)  [unwired: 14 in]
            n106 = call "CommonVIs_Wait.vi"("error in"=w272) -> ("error out"=w271:errorcluster)  [unwired: 9 in]
            n107 = disable-structure shown="Enabled" {
              disable-tunnel: [w292 w293] -> w270
              disable-tunnel: w273 -> [w291 _]
              disable-tunnel: w271 -> [w290 w293]
              frame Enabled {
                n108 = invoke class="LVClassLibrary" method="Save"(reference=w291, error in=w290) -> (error out=w292:errorcluster)  [unwired: 2 in, 3 out]
              }
              frame Disabled {
              }
            }
            n109 = Close Reference(reference=w269, error in (no error)=w270) -> ()  [unwired: 1 out]
          }
          frame "UpdateIcons" {
            n110 = Unbundle By Name(w328) -> ("ClassRefnum"=w327:refnum<vi>)
            n111 = Unbundle By Name(w328) -> ("SubClass"=w332:bool, "ClassName"=w329:string)
            n112 = call-dynamic "ProgressWindow.vi"("ClassWriter in"=w315, "Message(Exit)"="Hide", "error in (no error)"=w321) -> ("ClassWriter out"=w316:refnum<class "ClassWriterGOOP300.lvclass">, "error out"=w320:errorcluster)  [unwired: 15 in]
            n113 = Empty String/Path?(string/path=w326) -> (empty?=w325:bool)
            n114 = Not(x=w325) -> (.not. x?=w324:bool)
            n115 = call "GDSLvIcon_DialogUpdateClass.vi"("ClassPath(FilePath/ProjectTreePath/LvCLassRef)"=w327, "ClassName"=w329, "AutoUpdate"=w324, "error in (no error)"=w320, "HeaderToApply (take from VIRef or /use 2D-8bit header, Ignored if not wired)"=w326) -> ("error out"=w319:errorcluster)  [unwired: 11 in, 3 out]
            n116 = Select(t="GetDerivedClassConstructor", s=w332, f="AddFolders") -> (s? t:f=w330:string)
            n117 = call-dynamic "ProgressWindow.vi"("ClassWriter in"=w316, "Message(Exit)"="UnHide", "error in (no error)"=w319) -> ("error out"=w318:errorcluster)  [unwired: 15 in, 1 out]
          }
          frame "GetDerivedClassConstructor" {
            # "USE BASE CLASS PATH"
            n118 = Unbundle By Name(w350) -> ("ClassRefnum"=w348:refnum<vi>)
            n119 = property class="LVClassLibrary"(reference=w348, error in=w347) -> (error out=w344:errorcluster, "Parent"=w336:refnum<vi>)  [unwired: 1 out]
            n120 = property class="LVClassLibrary"(reference=w336, error in=w344) -> (reference out=w335:refnum<vi>, error out=w334:errorcluster, "Path"=w342:path)
            n121 = Strip Path(path=w342) -> (stripped path=w341:path)  [unwired: 1 out]
            n122 = call <vilib>:"Recursive File List.vi"("pattern"="*_Create.vi", "Treat LLBs as Folders?"=TRUE, "Folder Path"=w341) -> ("All Files in Dir"=w339:path[], "dup Folder Path"=w337:path)  [unwired: 4 in, 3 out]
            n123 = Close Reference(reference=w335, error in (no error)=w334) -> (error out=w333:errorcluster)
            n124 = Array Size(array=w339) -> (size(s)=w340:i32)
            n125 = case shown="0" w340 {
              tunnel: w339 -> [w352 _]
              tunnel: [w352 w353] -> w338
              tunnel: w337 -> [_ w354]
              frame Default {
              }
              frame 0 {
                n126 = call <vilib>:"Recursive File List.vi"("pattern"="*_Init.vi", "Treat LLBs as Folders?"=TRUE, "Folder Path"=w354) -> ("All Files in Dir"=w353:path[])  [unwired: 4 in, 4 out]
              }
            }
            n127 = Index Array(array=w338) -> (element=w343:path)  [unwired: 1 in]
            n128 = Bundle By Name(cluster=w350, "BaseConstructorBase"=w343) -> (w351:T5)
          }
          frame "UpdateVIs" {
            (unwired) "AnyProtectedAttributesToUpdate?"
            # "This is a sub class, replace all BaseClass References with Select base class.\nIf base not equal to root, also replace BaseClass ObjectRef with Root-Base ObjectRef"
            n129 = Unbundle By Name(w364) -> ("TemplBaseConstructorBase"=w361:path, "BaseConstructorBase"=w357:path)
            n130 = Unbundle By Name(w364) -> ("VIs"=w377:refnum<vi>[])
            n131 = call "CreateVINamesToReplace.vi"("Foldername"="utils" ("name or relative path"), "NewVIName"="_New.vi" ("string"), "BaseConstructorBase"=w357, "TemplBaseConstructorBase"=w361) -> ("NewVIName"=w372:path, "OldVIName"=w373:path)  [unwired: 5 in]
            n132 = call "CreateVINamesToReplace.vi"("NewVIName"="_Init.vi" ("string"), "BaseConstructorBase"=w357, "TemplBaseConstructorBase"=w361) -> ("NewVIName"=w368:path, "OldVIName"=w369:path)  [unwired: 6 in]
            n133 = call "CreateVINamesToReplace.vi"("NewVIName"="_CleanUp.vi" ("string"), "BaseConstructorBase"=w357, "TemplBaseConstructorBase"=w361) -> ("NewVIName"=w365:path, "OldVIName"=w366:path)  [unwired: 6 in]
            n134 = call "CreateVINamesToReplace.vi"("NewVIName"="_GOOPKernel.vi" ("string"), "BaseConstructorBase"=w357, "TemplBaseConstructorBase"=w361) -> ("NewVIName"=w358:path, "OldVIName"=w359:path)  [unwired: 6 in]
            n135 = for {
              shift-right: [w408] -> w362
              shift-left: w376 -> [w405]
              tunnel: w377 -> [w399] mode=indexing
              tunnel: w361 -> [w407]
              tunnel: w357 -> [w406]
              tunnel: w373 -> [w398]
              tunnel: w372 -> [w397]
              tunnel: w369 -> [w391]
              tunnel: w368 -> [w390]
              tunnel: w366 -> [w386]
              tunnel: w365 -> [w385]
              tunnel: w359 -> [w384]
              tunnel: w358 -> [w383]
              n136 = property class="VI"(reference=w399) -> ("Name"=w380:string)  [unwired: 1 in, 2 out]
              n137 = Match Pattern(string=w380, regular expression="_Create.vi") -> (offset past match=w404:i32)  [unwired: 1 in, 3 out]
              n138 = Match Pattern(string=w380, regular expression="_New.vi") -> (offset past match=w402:i32)  [unwired: 1 in, 3 out]
              n139 = Match Pattern(string=w380, regular expression="_Init.vi") -> (offset past match=w395:i32)  [unwired: 1 in, 3 out]
              n140 = Match Pattern(string=w380, regular expression="_CleanUp.vi") -> (offset past match=w388:i32)  [unwired: 1 in, 3 out]
              n141 = Match Pattern(string=w380, regular expression="_GOOPKernel.vi") -> (offset past match=w382:i32)  [unwired: 1 in, 3 out]
              n142 = Greater Or Equal To 0?(x=w404) -> (x >= 0?=w393:bool)
              n143 = Greater Or Equal To 0?(x=w402) -> (x >= 0?=w401:bool)
              n144 = Greater Or Equal To 0?(x=w395) -> (x >= 0?=w392:bool)
              n145 = Greater Or Equal To 0?(x=w388) -> (x >= 0?=w387:bool)
              n146 = Greater Or Equal To 0?(x=w382) -> (x >= 0?=w379:bool)
              n147 = Compound Arithmetic op=OR(w393, w401, w392, w387, w379) -> (w400:bool)
              n148 = case shown="True" w400 {
                tunnel: w405 -> [w409 w428]
                tunnel: [w409 w427] -> w408
                tunnel: w399 -> [_ w426]
                tunnel: w407 -> [_ w424]
                tunnel: w406 -> [_ w423]
                tunnel: w401 -> [_ w425]
                tunnel: w398 -> [_ w420]
                tunnel: w397 -> [_ w419]
                tunnel: w392 -> [_ w418]
                tunnel: w391 -> [_ w417]
                tunnel: w390 -> [_ w416]
                tunnel: w387 -> [_ w415]
                tunnel: w386 -> [_ w414]
                tunnel: w385 -> [_ w413]
                tunnel: w384 -> [_ w412]
                tunnel: w383 -> [_ w411]
                tunnel: w379 -> [_ w410]
                frame False {
                }
                frame True {
                  n149 = case shown="False" w425 {
                    tunnel: w424 -> [w440 _]
                    tunnel: w423 -> [w438 _]
                    tunnel: [w439 w468] -> w422
                    tunnel: [w437 w467] -> w421
                    tunnel: w420 -> [_ w468]
                    tunnel: w419 -> [_ w467]
                    tunnel: w418 -> [w441 _]
                    tunnel: w417 -> [w436 _]
                    tunnel: w416 -> [w435 _]
                    tunnel: w415 -> [w434 _]
                    tunnel: w414 -> [w433 _]
                    tunnel: w413 -> [w432 _]
                    tunnel: w412 -> [w431 _]
                    tunnel: w411 -> [w430 _]
                    tunnel: w410 -> [w429 _]
                    frame False {
                      n150 = case shown="False" w441 {
                        tunnel: w440 -> [w450 _]
                        tunnel: [w447 w466] -> w439
                        tunnel: w438 -> [w448 _]
                        tunnel: [w449 w465] -> w437
                        tunnel: w436 -> [_ w466]
                        tunnel: w435 -> [_ w465]
                        tunnel: w434 -> [w451 _]
                        tunnel: w433 -> [w446 _]
                        tunnel: w432 -> [w445 _]
                        tunnel: w431 -> [w444 _]
                        tunnel: w430 -> [w443 _]
                        tunnel: w429 -> [w442 _]
                        frame False {
                          n151 = case shown="False" w451 {
                            tunnel: [w457 w464] -> w447
                            tunnel: w450 -> [w458 _]
                            tunnel: [w456 w463] -> w449
                            tunnel: w448 -> [w455 _]
                            tunnel: w446 -> [_ w464]
                            tunnel: w445 -> [_ w463]
                            tunnel: w444 -> [w454 _]
                            tunnel: w443 -> [w453 _]
                            tunnel: w442 -> [w452 _]
                            frame False {
                              n152 = case shown="True" w452 {
                                tunnel: w458 -> [w460 _]
                                tunnel: [w460 w462] -> w457
                                tunnel: [w459 w461] -> w456
                                tunnel: w455 -> [w459 _]
                                tunnel: w454 -> [_ w462]
                                tunnel: w453 -> [_ w461]
                                frame False {
                                }
                                frame True {
                                }
                              }
                            }
                            frame True {
                            }
                          }
                        }
                        frame True {
                        }
                      }
                    }
                    frame True {
                    }
                  }
                  n153 = while {
                    tunnel: w428 -> [w482]
                    tunnel: [w479] -> w427
                    tunnel: w426 -> [w469]
                    tunnel: w421 -> [w470]
                    tunnel: w422 -> [w471]
                    i -> [w481]
                    stop <- w480 continue-if-true
                    n154 = File/Directory Info(path=w471) -> (error out=w473:errorcluster)  [unwired: 1 in, 6 out]
                    n155 = File/Directory Info(path=w470) -> (error out=w474:errorcluster)  [unwired: 1 in, 6 out]
                    n156 = Unbundle By Name(w473) -> ("status"=w477:bool)
                    n157 = Unbundle By Name(w474) -> ("status"=w478:bool)
                    n158 = Empty String/Path?(string/path=w470) -> (empty?=w476:bool)
                    n159 = Empty String/Path?(string/path=w471) -> (empty?=w475:bool)
                    n160 = Compound Arithmetic op=AND(invert w477, invert w475, invert w478, invert w476) -> (w472:bool)
                    n161 = case shown="True" w472 {
                      tunnel: w482 -> [w483 w495]
                      tunnel: w470 -> [_ w494]
                      tunnel: w471 -> [_ w493]
                      tunnel: w481 -> [_ w491]
                      tunnel: [_ w488] -> w480
                      tunnel: w469 -> [_ w487]
                      tunnel: [w483 w484] -> w479
                      frame False {
                      }
                      frame True {
                        n162 = Build Array(w493) -> (w486:path[])
                        n163 = Build Array(w494) -> (w485:path[])
                        n164 = call "Scripting_ReplaceVisAndControls.vi"("ViRef"=w487, "OldVIsAndControls"=w486, "NewVIsAndControls"=w485, "error in (no error)"=w495) -> ("error out"=w484:errorcluster)  [unwired: 14 in, 1 out]
                        n165 = Unbundle By Name(w484) -> ("status"=w492:bool)  [unwired: 1 out]
                        n166 = Less Or Equal?(x=w491, y=3) -> (x <= y?=w489:bool)
                        n167 = And(x=w489, y=w492) -> (x .and. y?=w488:bool)
                      }
                    }
                  }
                }
              }
            }
            n168 = Unbundle By Name(w364) -> ("TempClass"=w363:refnum<vi>)
            n169 = stacked-sequence {
              tunnel: w363 -> [w378]
              tunnel: w362 -> [_]
              frame #0 {
                n170 = Close Reference(reference=w378) -> ()  [unwired: 1 in, 1 out]
              }
            }
          }
          frame "AnyProtectedAttributesToUpdate?" {
            n171 = Unbundle By Name(w497) -> ("BaseClassFolder"=w515:path)
            n172 = Unbundle By Name(w497) -> ("VIs"=w520:refnum<vi>[])
            n173 = call <vilib>:"Recursive File List.vi"("Folder Path"=w515) -> ("All Files in Dir"=w504:path[])  [unwired: 6 in, 4 out]
            n174 = for {
              tunnel: w520 -> [w548] mode=indexing
              tunnel: [w547] -> w501 mode=indexing
              tunnel: [w545] -> w517 mode=indexing
              n175 = property class="VI"(reference=w548) -> ("Path"=w547:path)  [unwired: 1 in, 2 out]
              n176 = Strip Path(path=w547) -> (name=w546:string)  [unwired: 1 out]
              n177 = To Lower Case(string=w546) -> (all lower case string=w545:string)
            }
            n178 = for {
              tunnel: w504 -> [w533] mode=indexing
              tunnel: [w532] -> w510 mode=indexing
              n179 = Strip Path(path=w533) -> (name=w534:string)  [unwired: 1 out]
              n180 = To Lower Case(string=w534) -> (all lower case string=w532:string)
            }
            n181 = To Lower Case(string="ObjectAttributes.ctl") -> (all lower case string=w514:string)
            n182 = Unbundle By Name(w497) -> ("App"=w496:refnum<vi>)
            n183 = To Lower Case(string="ClassAttributes.ctl") -> (all lower case string=w509:string)
            n184 = Search 1D Array(1D array=w510, element=w514) -> (index of element=w505:i32)  [unwired: 1 in]
            n185 = Search 1D Array(1D array=w510, element=w509) -> (index of element=w503:i32)  [unwired: 1 in]
            n186 = Search 1D Array(1D array=w517, element=w514) -> (index of element=w506:i32)  [unwired: 1 in]
            n187 = Search 1D Array(1D array=w517, element=w509) -> (index of element=w500:i32)  [unwired: 1 in]
            n188 = Greater Or Equal To 0?(x=w503) -> (x >= 0?=w508:bool)
            n189 = Greater Or Equal To 0?(x=w505) -> (x >= 0?=w512:bool)
            n190 = Greater Or Equal To 0?(x=w506) -> (x >= 0?=w513:bool)
            n191 = Greater Or Equal To 0?(x=w500) -> (x >= 0?=w507:bool)
            n192 = And(x=w512, y=w513) -> (x .and. y?=w511:bool)
            n193 = And(x=w508, y=w507) -> (x .and. y?=w502:bool)
            n194 = case shown="True" w511 {
              tunnel: w518 -> [w543 w544]
              tunnel: w501 -> [w542 _]
              tunnel: w504 -> [w540 _]
              tunnel: w506 -> [w538 _]
              tunnel: w505 -> [w537 _]
              tunnel: [w536 w544] -> w499
              tunnel: w496 -> [w535 _]
              frame True {
                n195 = Index Array(array=w542, index=w538) -> (element=w541:path)
                n196 = Index Array(array=w540, index=w537) -> (element=w539:path)
                n197 = call "Scripting_UpdateProtectedClassData.vi"("AppRef"=w535, "error in (no error)"=w543, "NewBaseAttribute"=w539, "BaseAttribute"=w541) -> ("error out"=w536:errorcluster)  [unwired: 6 in, 1 out]
              }
              frame False {
              }
            }
            n198 = case shown="True" w502 {
              tunnel: w501 -> [w530 _]
              tunnel: w504 -> [w528 _]
              tunnel: w500 -> [w526 _]
              tunnel: w503 -> [w525 _]
              tunnel: w499 -> [w524 w531]
              tunnel: [w523 w531] -> w498
              tunnel: w496 -> [w522 _]
              frame True {
                n199 = Index Array(array=w530, index=w526) -> (element=w529:path)
                n200 = Index Array(array=w528, index=w525) -> (element=w527:path)
                n201 = call "Scripting_UpdateProtectedClassData.vi"("AppRef"=w522, "error in (no error)"=w524, "NewBaseAttribute"=w527, "BaseAttribute"=w529) -> ("error out"=w523:errorcluster)  [unwired: 6 in, 1 out]
              }
              frame False {
              }
            }
          }
          frame "AddFolders" {
            n202 = Unbundle By Name(w554) -> ("ClassRefnum"=w565:refnum<vi>)
            n203 = Unbundle By Name(w554) -> ("TemplateName"=w564:string)
            n204 = Unbundle By Name(w552) -> ("ParentInterfaces"=w549:path[])
            n205 = call "UpdateClassApperance.vi"("ClassRefIn"=w565, "error in (no error)"=w566) -> ("ClassRefOut"=w550:refnum<vi>, "error out"=w560:errorcluster)  [unwired: 16 in]
            n206 = call "SetParentInterfaces.vi"("error in"=w560, "Parent Interfaces(ClassRef/Path)"=w549, "Class/InterfaceRefIn"=w550) -> ("error out"=w551:errorcluster)  [unwired: 7 in, 1 out]
            n207 = Unbundle By Name(w554) -> ("SubClass"=w555:bool)
            n208 = disable-structure shown="Enabled" {
              disable-tunnel: [w571 w573] -> w559
              disable-tunnel: [w569 _] -> w558
              disable-tunnel: w551 -> [w568 w573]
              frame Disabled {
                n209 = call "GOOP400_ConfigurationMemory.vi"("error in (no error)"=w568, "Action"=enum16{"Read", "Load", "Save"}."Read") -> ("OptionsOut"=w570:T13, "error out"=w571:errorcluster)  [unwired: 16 in]
                n210 = Unbundle By Name(w570) -> ("FlatFolderStructure"=w569:bool)
              }
              frame Enabled {
              }
            }
            n211 = Match Pattern(string=w564, regular expression="Interface") -> (offset past match=w562:i32)  [unwired: 1 in, 3 out]
            n212 = Greater Or Equal To 0?(x=w562) -> (x >= 0?=w561:bool)
            n213 = case shown="False" w561 {
              tunnel: [w579 w589] -> w567
              tunnel: w559 -> [w577 w589]
              tunnel: w565 -> [w576 _]
              tunnel: w558 -> [w575 _]
              frame False {
                (unwired) TRUE ("CreateThePfysicalFolderIfPossible(False)")
                n214 = Not(x=w575) -> (.not. x?=w574:bool)
                n215 = call "GDSProject_CreateFolder.vi"("Project Item To Create Folder Below(Use MyComputer if not wired)"=w576, "FolderName"="private", "error in (no error)"=w577, "CreateThePhysicalFolderIfPossible(False)"=w574) -> ("ItemOut"=w582:refnum<vi>, "FolderCreated"=w578:bool, "error out"=w580:errorcluster)  [unwired: 12 in, 1 out]
                n216 = case shown="True" w578 {
                  tunnel: w582 -> [_ w584]
                  tunnel: w580 -> [w583 w587]
                  tunnel: [w583 w585] -> w579
                  tunnel: w576 -> [_ w586]
                  frame False {
                  }
                  frame True {
                    n217 = invoke class="LVClassLibrary" method="Set Source Scope"(reference=w586, error in=w587, "SourceRef"=w584, "Scope"=T8."private" ("scope")) -> (error out=w585:errorcluster)  [unwired: 1 in, 4 out]
                    n218 = Close Reference(reference=w584, error in (no error)=w585) -> ()  [unwired: 1 out]
                  }
                }
              }
              frame True {
              }
            }
            n219 = Select(t="ReplaceBaseTemplateReferences", s=w555, f="UpdateObjectRefEnum") -> (s? t:f=w553:string)
          }
          frame "UpdateObjectRefEnum" {
            w629 = refnum<vi> refnum  # Enum
            w632 = refnum<vi> refnum  # TypedRefNum
            n220 = Unbundle By Name(w591) -> ("App"=w594:refnum<vi>, "ClassFolder"=w595:path)
            n221 = Unbundle By Name(w591) -> ("ClassName"=w598:string)
            n222 = Build Path(base path=w595, name or relative path="ObjectReference.ctl") -> (appended path=w601:path)
            n223 = call "Scripting_OpenViRef.vi"("error in"=w592, "ViPath/ViName/Viref"=w601, "AppRef"=w594) -> ("error out"=w613:errorcluster, "vi reference"=w614:refnum<vi>)  [unwired: 6 in, 1 out]
            n224 = invoke on="Save" class="VI" method="VI Icon.Get as Image Data"(reference=w614, error in=w613) -> (reference out=w612:refnum<vi>, error out=w611:errorcluster, "ImageData"=w610:T14)  [unwired: 4 in, 3 out]
            n225 = Unbundle By Name(w610) -> ("colors"=w607:u32[], "image"=w609:u8[])
            n226 = Delete From Array(array=w609, length=100, index=33) -> (deleted portion=w600:u8[])  [unwired: 1 out]
            n227 = property on="Panel" class="VI"(reference=w612, error in=w611) -> (reference out=w618:refnum<vi>, error out=w596:errorcluster, "Front Panel"=w597:refnum<vi>)
            n228 = property on="Ctrls" class="Pnl"(reference=w597, error in=w596) -> ("Controls[]"=w634:refnum<vi>[])  [unwired: 2 out]
            n229 = while {
              tunnel: w600 -> [w636] mode=indexing
              tunnel: [w636] -> w599
              i -> [w640]
              stop <- w637 continue-if-true
              w639 = 255
              n230 = Equal?(x=w636, y=w639) -> (x = y?=w641:bool)
              n231 = Less?(x=w640, y=w639) -> (x < y?=w638:bool)
              n232 = And(x=w641, y=w638) -> (x .and. y?=w637:bool)
            }
            n233 = Index Array(array=w634) -> (element=w633:refnum<vi>)  [unwired: 1 in]
            n234 = To More Specific Class(target class=w632, reference=w633, error in=w596) -> (specific class reference=w631:refnum<vi>, error out=w626:errorcluster)
            n235 = Build Array(w598) -> (w627:string[])
            n236 = property on="Ctrls" class="TypRef"(reference=w631, error in=w626) -> (reference out=w620:refnum<vi>, error out=w625:errorcluster, "Element"=w630:refnum<vi>)
            n237 = Index Array(array=w607, index=w599) -> (element=w604:u32)
            n238 = To More Specific Class(target class=w629, reference=w630, error in=w625) -> (specific class reference=w628:refnum<vi>, error out=w624:errorcluster)
            n239 = Equal To 0?(x=w604) -> (x = 0?=w605:bool)
            n240 = Select(t=u32 16777216, s=w605, f=w604) -> (s? t:f=w603:u32)
            n241 = property on="Ctrls" class="Enum"(reference=w628, error in=w624, "Strings []"=w627, "Named Numeric Colors:BG Color"=w603) -> (reference out=w623:refnum<vi>, error out=w622:errorcluster)
            n242 = Close Reference(reference=w623, error in (no error)=w622) -> (error out=w621:errorcluster)
            n243 = Close Reference(reference=w620, error in (no error)=w621) -> (error out=w619:errorcluster)
            n244 = Close Reference(reference=w597, error in (no error)=w619) -> (error out=w617:errorcluster)
            n245 = invoke on="Save" class="VI" method="Save.Instrument"(reference=w618, error in=w617) -> (reference out=w616:refnum<vi>, error out=w615:errorcluster)  [unwired: 4 in, 4 out]
            n246 = Close Reference(reference=w616, error in (no error)=w615) -> (error out=w593:errorcluster)
          }
          frame "ReplaceBaseTemplateReferences" {
            w651 = "ObjectReference.ctl" ("name or relative path")
            # "This is a sub class, replace all BaseClass References with Select base class.\nIf base not equal to root, also replace BaseClass ObjectRef with Root-Base ObjectRef"
            n247 = Unbundle By Name(w643) -> ("VIs"=w646:refnum<vi>[], "BaseClassFolder"=w644:path, "BaseClassName"=w645:string)  [unwired: 4 out]
            n248 = Unbundle By Name(w643) -> ("RootBaseClassFolder"=w659:path)
            n249 = Unbundle By Name(w643) -> ("TemplateParentName"=w658:string)
            n250 = call-dynamic "GetTemplatePath.vi"("reference in"=w649, "ClassTemplateSubDirectory"=w658) -> ("FolderPathOut"=w655:path)  [unwired: 13 in, 4 out]
            n251 = Build Path(base path=w655, name or relative path=w651) -> (appended path=w654:path)
            n252 = Build Path(base path=w659, name or relative path=w651) -> (appended path=w650:path)
            n253 = call "GOOP300_FindFilesToExchange.vi"("OldClassName(Prefix or suffix for some VIs)"=w658, "OldFolderPath"=w655, "NewFolderPath"=w644, "NewClassName(Prefix or suffix for some VIs)"=w645) -> ("OldFiles"=w653:path[], "NewFileArray"=w652:path[])  [unwired: 14 in]
            n254 = Build Array (concatenate)(w654, w653) -> (w656:path[])
            n255 = Build Array (concatenate)(w650, w652) -> (w657:path[])
            n256 = for {
              tunnel: w646 -> [w664] mode=indexing
              shift-right: [w662] -> w648
              shift-left: w647 -> [w663]
              tunnel: w656 -> [w661]
              tunnel: w657 -> [w660]
              n257 = call "Scripting_ReplaceVisAndControls.vi"("ViRef"=w664, "OldVIsAndControls"=w661, "NewVIsAndControls"=w660, "error in (no error)"=w663) -> ("error out"=w662:errorcluster)  [unwired: 14 in, 1 out]
            }
          }
          frame "PlaceRefInAttribute" {
            n258 = Unbundle By Name(w669) -> ("ClassRefnum"=w670:refnum<vi>)
            n259 = Unbundle By Name(w669) -> ("SubClass"=w666:bool, "RootBaseClassFolder"=w673:path)
            n260 = Unbundle By Name(w669) -> ("LvClassFolderPath"=w671:path)
            n261 = Select(t=w673, s=w666, f=w671) -> (s? t:f=w672:path)
            n262 = case shown="True" w666 {
              tunnel: w672 -> [_ w678]
              tunnel: w670 -> [_ w677]
              tunnel: w668 -> [w674 w676]
              tunnel: [w674 w675] -> w667
              frame False {
              }
              frame True {
                n263 = call "Scripting_PlaceGoopRefInClassAttribute.vi"("error in"=w676, "ObjectRef_LvClassFolderPath"=w678, "ClassRefnum"=w677) -> ("error out"=w675:errorcluster)  [unwired: 1 in, 3 out]
              }
            }
          }
          frame "ReentrantDestructor?" {
            # "Use reentrant if this is a base class.\nor this is a sub class with a reentrant base class destructor"
            n264 = Unbundle By Name(w680) -> ("App"=w683:refnum<vi>, "BaseClassName"=w682:string, "VIs"=w684:refnum<vi>[])
            n265 = for {
              tunnel: w684 -> [w694] mode=indexing
              tunnel: w682 -> [w689]
              tunnel: w683 -> [w688]
              n266 = property class="VI"(reference=w694) -> (reference out=w690:refnum<vi>, "Name"=w693:string)  [unwired: 1 in, 1 out]
              n267 = Match Pattern(string=w693, regular expression=":Destroy\\2E[Vv][Ii]$") -> (offset past match=w691:i32)  [unwired: 1 in, 3 out]
              n268 = case shown="Default" w691 {
                tunnel: w690 -> [w699 _]
                tunnel: w689 -> [w698 _]
                tunnel: w688 -> [w695 _]
                frame Default {
                  n269 = case shown="\"False\", Default" w698 {
                    selector: w698 -> [w710 _]
                    tunnel: [w701 TRUE] -> w697
                    tunnel: w695 -> [w700 _]
                    frame "False", Default {
                      n270 = Concatenate Strings(w710, ".lvclass:Destroy.vi" ("regular expression")) -> (w708:string)
                      n271 = call "Scripting_OpenViRef.vi"("ViPath/ViName/Viref"=w708, "AppRef"=w700) -> ("error out"=w706:errorcluster, "vi reference"=w707:refnum<vi>)  [unwired: 7 in, 1 out]
                      n272 = property class="VI"(reference=w707, error in=w706) -> (reference out=w705:refnum<vi>, error out=w704:errorcluster, "Exec.IsReentrant"=w702:bool)
                      n273 = Unbundle(w704) -> ("status"=w703:bool)  [unwired: 2 out]
                      n274 = Close Reference(reference=w705, error in (no error)=w704) -> ()  [unwired: 1 out]
                      n275 = Or(x=w703, y=w702) -> (x .or. y?=w701:bool)
                    }
                    frame "" {
                    }
                  }
                  n276 = property class="VI"(reference=w699, "Exec.IsReentrant"=w697, "Exec.ReentrancyType"=T9."Share clones between instances" ("Execution:Reentrancy Type")) -> ()  [unwired: 1 in, 2 out]
                }
                frame -1 {
                }
              }
            }
            n277 = Unbundle By Name(w680) -> ("llb"=w679:bool)
            n278 = case shown="False" w679 {
              tunnel: ["CloseRefs" "ConvertToLLb"] -> w685
              frame False {
              }
              frame True {
              }
            }
          }
          frame "ConvertToLLb" {
            n279 = Unbundle By Name(w728) -> ("ClassFolder"=w713:path)
            n280 = Unbundle By Name(w728) -> ("VIs"=w730:refnum<vi>[])
            n281 = Unbundle By Name(w728) -> ("ClassRefnum"=w727:refnum<vi>)
            n282 = Unbundle By Name(w733) -> ("ClassFolder"=w732:path)
            n283 = call <vilib>:"New VI Library.vi"("error in (no error)"=w731, "VI library path in"=w732) -> ("error out"=w729:errorcluster, "VI library path out"=w725:path)  [unwired: 8 in]
            n284 = for {
              tunnel: w730 -> [w747] mode=indexing
              tunnel: w725 -> [w744]
              shift-right: [w738] -> w715
              shift-left: w729 -> [w743]
              tunnel: w713 -> [w736]
              n285 = property class="VI"(reference=w747, error in=w743) -> (reference out=w746:refnum<vi>, error out=w742:errorcluster, "Path"=w745:path)
              n286 = Strip Path(path=w745) -> (stripped path=w737:path, name=w741:string)
              n287 = Build Path(base path=w744, name or relative path=w741) -> (appended path=w740:path)
              n288 = Equal?(x=w737, y=w736) -> (x = y?=w735:bool)
              n289 = invoke class="VI" method="Save.Instrument"(reference=w746, error in=w742, "Path to saved file"=w740) -> (error out=w739:errorcluster)  [unwired: 3 in, 5 out]
              n290 = case shown="True" w735 {
                tunnel: w740 -> [_ w752]
                tunnel: w739 -> [w748 w751]
                tunnel: [w748 w750] -> w738
                frame False {
                }
                frame True {
                  n291 = call <vilib>:"Librarian Get Info.vi"("error in (no error)"=w751, "path"=w752) -> ("error out"=w753:errorcluster, "file information"=w755:T15, "dup path"=w756:path)  [unwired: 7 in]
                  n292 = Bundle By Name(cluster=w755, "top level"=TRUE) -> (w754:T15)
                  n293 = call <vilib>:"Librarian Set Info.vi"("error in (no error)"=w753, "file information"=w754, "path"=w756) -> ("error out"=w750:errorcluster)  [unwired: 7 in, 1 out]
                }
              }
            }
            n294 = property class="LVClassLibrary"(reference=w727, error in=w715) -> (reference out=w723:refnum<vi>, "Path"=w726:path)  [unwired: 1 out]
            n295 = Strip Path(path=w726) -> (name=w724:string)  [unwired: 1 out]
            n296 = Build Path(base path=w725, name or relative path=w724) -> (appended path=w717:path)
            n297 = invoke class="LVClassLibrary" method="Save"(reference=w723, "Path"=w717) -> (error out=w716:errorcluster)  [unwired: 2 in, 3 out]
            n298 = call <vilib>:"Librarian Get Info.vi"("error in (no error)"=w716, "path"=w717) -> ("error out"=w721:errorcluster, "file information"=w719:T15, "dup path"=w718:path)  [unwired: 7 in]
            n299 = Bundle By Name(cluster=w719, "top level"=TRUE) -> (w720:T15)
            n300 = call <vilib>:"Librarian Set Info.vi"("error in (no error)"=w721, "file information"=w720, "path"=w718) -> ("error out"=w714:errorcluster)  [unwired: 7 in, 1 out]
            n301 = Delete(path (use dialog)=w713, entire hierarchy (F)=TRUE, error in=w714) -> ()  [unwired: 2 in, 3 out]
          }
          frame "CloseRefs", "Error", Default {
            n302 = case shown="\"CloseRefs\"" w775 {
              tunnel: w776 -> [w798 w806]
              tunnel: w759 -> [w797 w802]
              tunnel: [w798 w805] -> w760
              frame "False", Default {
                n303 = Unbundle By Name(w797) -> ("VIs"=w796:refnum<vi>[])
                n304 = Close Reference(reference=w796) -> ()  [unwired: 1 in, 1 out]
              }
              frame "CloseRefs" {
                n305 = Unbundle By Name(w802) -> ("ClassRefnum"=w801:refnum<vi>)
                n306 = Unbundle By Name(w802) -> ("ViLocked"=w804:bool[], "VIs"=w807:refnum<vi>[])
                n307 = Unbundle By Name(w802) -> ("ClassSettings"=w803:T2)
                n308 = call "GDSLvClass_StoreClassType.vi"("Class Refnum In"=w801, "ClassSettings"=w803, "CheckAndFixConnectorPaneType(False)"=TRUE) -> ("error out"=w799:errorcluster)  [unwired: 15 in, 1 out]
                n309 = for {
                  tunnel: w807 -> [w812] mode=indexing
                  shift-right: [w808] -> w805
                  shift-left: w806 -> [w813]
                  tunnel: w804 -> [w809] mode=indexing
                  tunnel: w799 -> [_]
                  n310 = case shown="True" w809 {
                    tunnel: w813 -> [w817 w823]
                    tunnel: w812 -> [w818 w822]
                    tunnel: [w817 w821] -> w811
                    tunnel: [w818 w820] -> w810
                    frame False {
                    }
                    frame True {
                      n311 = invoke class="VI" method="Lock State.Set"(reference=w822, error in=w823, "lockState"=T10."Locked (No Password)" ("Lock State")) -> (reference out=w820:refnum<vi>, error out=w821:errorcluster)  [unwired: 4 in, 5 out]
                    }
                  }
                  n312 = call "Scripting_SaveVi.vi"("ForceResaving(False)"=TRUE, "error in (no error)"=w811, "VIRefToSaveIn"=w810) -> ("error out"=w816:errorcluster, "VIRefToSaveOut"=w815:refnum<vi>)  [unwired: 7 in]
                  n313 = Close Reference(reference=w815, error in (no error)=w816) -> (error out=w808:errorcluster)
                }
              }
            }
            n314 = Unbundle By Name(w759) -> ("TempClass"=w758:refnum<vi>)
            n315 = stacked-sequence {
              tunnel: w760 -> [w778]
              tunnel: [w778] -> w757
              tunnel: w758 -> [w779]
              frame #0 {
                n316 = Close Reference(reference=w779) -> ()  [unwired: 1 in, 1 out]
              }
            }
            n317 = Unbundle By Name(w759) -> ("DeleteFiles"=w770:path[], "App"=w762:refnum<vi>, "ProjectRefnum"=w773:refnum<vi>, "ClassRefnum"=w769:refnum<vi>)
            n318 = call "GDSLvClass_SaveEverythingInClass.vi"("ClassRefIn"=w769, "error in"=w757) -> ("ClassRefOut"=w764:refnum<vi>, "error out"=w766:errorcluster)  [unwired: 16 in]
            n319 = case shown="False" w767 {
              tunnel: [w782 w783] -> w774
              tunnel: w766 -> [w781 w783]
              tunnel: w764 -> [w780 _]
              frame False {
                n320 = Close Reference(reference=w780, error in (no error)=w781) -> (error out=w782:errorcluster)
              }
              frame True {
              }
            }
            n321 = Close Reference(reference=w773, error in (no error)=w774) -> (error out=w763:errorcluster)
            n322 = Close Reference(reference=w762, error in (no error)=w763) -> (error out=w761:errorcluster)
            n323 = for {
              shift-right: [w794] -> w765
              shift-left: w761 -> [w795]
              tunnel: w770 -> [w793] mode=indexing
              tunnel: [w792] -> w768 mode=indexing
              n324 = Delete(path (use dialog)=w793, error in=w795) -> (error out=w794:errorcluster)  [unwired: 3 in, 2 out]
              n325 = Strip Path(path=w793) -> (stripped path=w792:path)  [unwired: 1 out]
            }
            n326 = for {
              tunnel: w768 -> [w788] mode=indexing
              n327 = List Folder(path=w788) -> (path out=w784:path, filenames=w787:string[], error out=w785:errorcluster)  [unwired: 3 in, 1 out]
              n328 = Empty Array?(array=w787) -> (empty?=w786:bool)
              n329 = case shown="True" w786 {
                tunnel: w785 -> [_ w791]
                tunnel: w784 -> [_ w790]
                tunnel: [_ w789] -> _
                frame False {
                }
                frame True {
                  n330 = Delete(path (use dialog)=w790, error in=w791) -> (error out=w789:errorcluster)  [unwired: 3 in, 2 out]
                }
              }
            }
            n331 = call "GDSError_LogErrorInformation.vi"("State"=w771, "LocalVariableData"=w759, "error in (no error)"=w765) -> ("error out"=w772:errorcluster)  [unwired: 16 in]
          }
        }
        n332 = Equal?(x=w34, y="Exit") -> (x = y?=w38:bool)
        n333 = Select(t="Error", s=w33, f=w34) -> (s? t:f=w37:string)
      }
      n334 = Unbundle By Name(w14) -> ("ClassRefnum"=w17:refnum<vi>, "TemplateVersion"=w16:string)
    }
    frame Error {
    }
  }
  "error out" <- w11
  "LVClassLibraryRefnum" <- w5
  "TemplateVersionUsed" <- w4
  "ClassWriterGOOP300.lvclass" <- "ClassWriterGOOP300.lvclass"
